vi "EDWARDS grappes.vi"() -> ()   [LabVIEW 2022 SP3]
uses:
  Variables globales/Variable glob Edwards.vi
panel:
  out "sortie d'erreur":errorcluster
  out "error out":errorcluster
  # "Lancement traitement valeurs grappes pour chaque grappe définie"
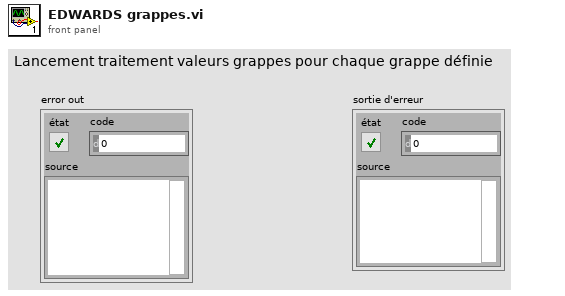
[diagram p1: front panel]
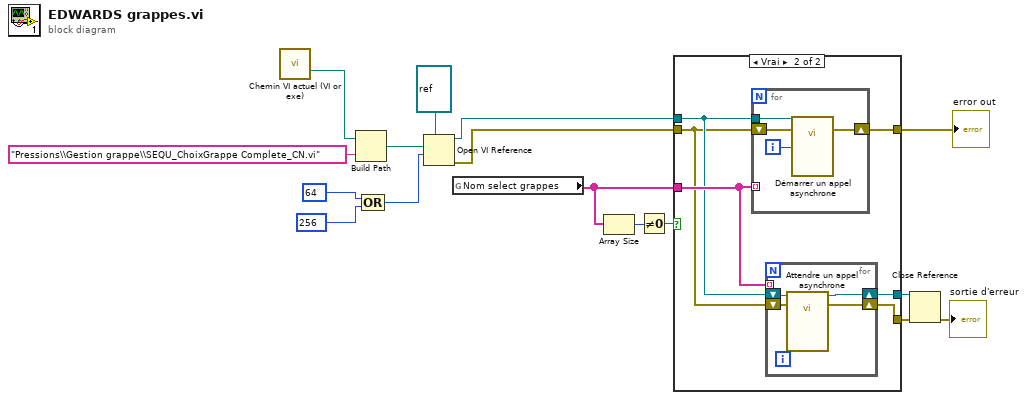
[diagram p0: block diagram]
diagram:
  n1 = call "Chemin VI actuel (VI or exe).vi"() -> ("VI or executable installation directory"=w1:path)  [unwired: 14 in, 1 out]
  n2 = Build Path(base path=w1, name or relative path="Pressions\\Gestion grappe\\SEQU_ChoixGrappe Complete_CN.vi" ("nom ou chemin relatif")) -> (appended path=w16:path)
  n3 = Compound Arithmetic op=OR(64 ("options"), 256 ("options")) -> (w12:i32)
  n4 = Open VI Reference(type specifier VI Refnum (for type only)=refnum<vi> refnum ("spécificateur de type du refnum de VI (pour type seulement)"), vi path=w16, options=w12) -> (vi reference=w10:refnum<vi>, error out=w9:errorcluster)  [unwired: 3 in]
  n5 = global read "Variable glob Edwards.vi" "Nom select grappes"() -> (w2:string[])
  n6 = Array Size(array=w2) -> (size(s)=w4:i32)
  n7 = Not Equal To 0?(x=w4) -> (x != 0?=w3:bool)
  n8 = case shown="Vrai" w3 {
    tunnel: w10 -> [w17 w20]
    tunnel: w9 -> [w18 w19]
    tunnel: [w18 w24] -> w8
    tunnel: [w17 w23] -> w7
    tunnel: [w18 w22] -> w6
    tunnel: w2 -> [_ w21]
    frame False {
    }
    frame True {
      n9 = for {
        tunnel: w21 -> [_] mode=indexing
        tunnel: w20 -> [w32]
        shift-right: [w29] -> w24
        shift-left: w19 -> [w30]
        i -> [w31]
        n10 = call-by-ref "Démarrer un appel asynchrone"(reference=w32, error in=w30, "indice grappe"=w31) -> (error out=w29:errorcluster)  [unwired: 2 in, 2 out]
      }
      n11 = for {
        tunnel: w21 -> [_] mode=indexing
        shift-right: [w27] -> w23
        shift-left: w20 -> [w28]
        shift-right: [w25] -> w22
        shift-left: w19 -> [w26]
        n12 = call-by-ref "Attendre un appel asynchrone"(reference=w28, error in=w26) -> (reference out=w27:refnum<vi>, error out=w25:errorcluster)  [unwired: 3 in, 1 out]
      }
    }
  }
  "error out" <- w8
  n13 = Close Reference(reference=w7, error in (no error)=w6) -> (error out=→"sortie d'erreur":errorcluster)
